vi "Configure the Function on 2nd Display.vi"(5 "Manual Range":dbl format="%#.9e", 7 "Enable Auto Range":bool=TRUE, 8 "error in":errorcluster, 10 "Function":u8(ring)=8 items=["DC Voltage", "AC Voltage", "DC Current", "AC Current", "2-Wire Resistance", "4-Wire Resistance", "Frequency", "Period", "None"], 11 "VISA resource name":refnum<visa-resource-name>) -> (0 "error out":errorcluster, 3 "VISA resource name out":refnum<visa-resource-name>)   [LabVIEW 2012, in "GDM-9052.lvlib"]
uses:
  GDM-9052.lvlib
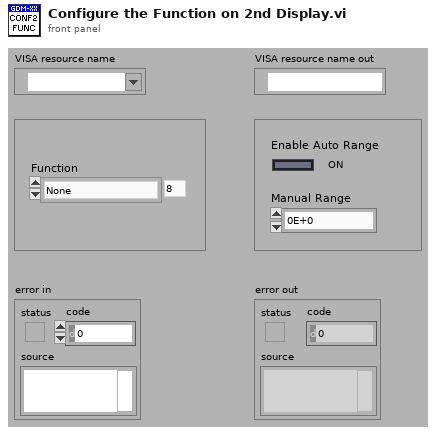
[diagram p1: front panel]
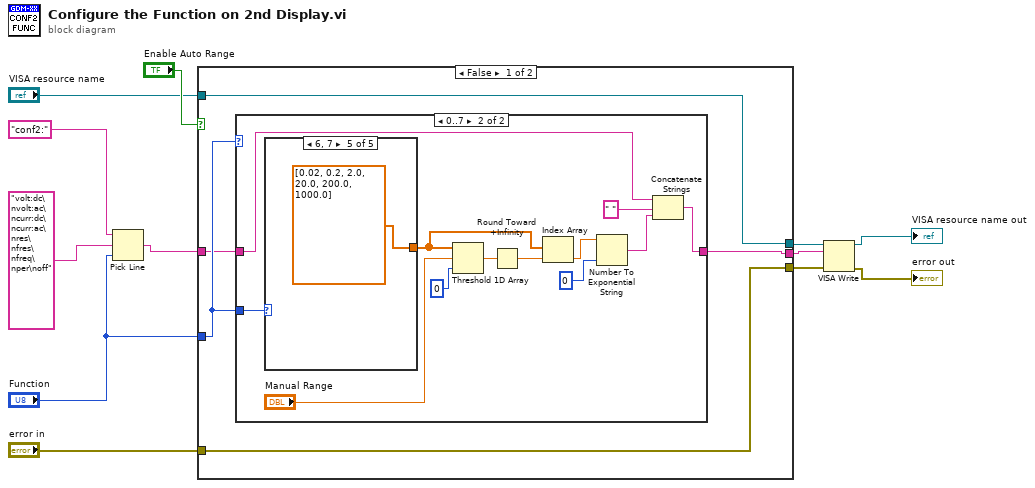
[diagram p0: block diagram]
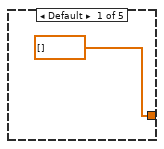
[diagram p3: hidden frame]
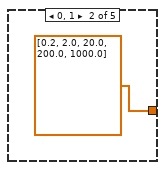
[diagram p4: hidden frame]
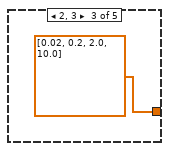
[diagram p5: hidden frame]
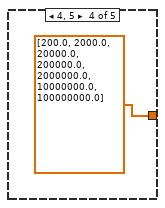
[diagram p6: hidden frame]
diagram:
  n1 = Pick Line(string ("")="conf2:", multi-line string="volt:dc\nvolt:ac\ncurr:dc\ncurr:ac\nres\nfres\nfreq\nper\noff", line index="Function") -> (output string=w8:string)
  n2 = case shown="False" "Enable Auto Range" {
    tunnel: "Function" -> [w17 _]
    tunnel: w8 -> [w16 w36]
    tunnel: "VISA resource name" -> [w13 w38]
    tunnel: "error in" -> [w14 w37]
    tunnel: [w13 w38] -> w2
    tunnel: [w14 w37] -> w1
    tunnel: [w15 w36] -> w5
    frame False {
      n3 = case shown="0..7" w17 {
        tunnel: w17 -> [_ w19]
        tunnel: w16 -> [w18 w21]
        tunnel: [w18 w20] -> w15
        frame Default {
        }
        frame 0..7 {
          n4 = case shown="6, 7" w19 {
            tunnel: [dbl[] [] dbl[] [0.2, 2.0, 20.0, 200.0, 1000.0] dbl[] [0.02, 0.2, 2.0, 10.0] dbl[] [200.0, 2000.0, 20000.0, 200000.0, 2000000.0, 10000000.0, 100000000.0] dbl[] [0.02, 0.2, 2.0, 20.0, 200.0, 1000.0]] -> w26
            frame Default {
            }
            frame 0, 1 {
            }
            frame 2, 3 {
            }
            frame 4, 5 {
            }
            frame 6, 7 {
            }
          }
          n5 = Threshold 1D Array(1:0 ("start index (0)"), 2:"Manual Range", 3:w26) -> (0:w28:dbl)
          n6 = Round Toward +Infinity(x=w28) -> (ceil(x): smallest int >= x=w27:dbl)
          n7 = Index Array(array=w26, index=w27) -> (element=w25:dbl)
          n8 = Number To Exponential String(number=w25, precision (6)=i16 0) -> (E-format string=w22:string)  [unwired: 2 in]
          n9 = Concatenate Strings(w21, " " ("string"), w22) -> (w20:string)
        }
      }
    }
    frame True {
    }
  }
  n10 = VISA Write(VISA resource name=w2, write buffer=w5, error in (no error)=w1) -> (VISA resource name out=→"VISA resource name out":refnum<visa-resource-name>, error out=→"error out":errorcluster)  [unwired: 1 out]
